vi "Toast With Reply.vi"(8 "error in":errorcluster) -> (0 "error out":errorcluster, 3 "Toast XML":string)   [LabVIEW 2026]
doc: "Receive a text reply from a Windows toast as a LabVIEW User Event. Type a reason, click Send and inspect the Reason entry in Activation.User Inputs. An empty reply still returns the Reason key. Press Stop to close the example."
uses:
  ToastNotification/Activation.ctl
  ToastNotification/Argument.ctl
  PlugIns/UserEventActivationHandler/UserEventActivationHandler.lvclass
  PlugIns/UserEventActivationHandler/UserEventActivationHandler.lvclass/UserEventActivationHandler.ctl
  PlugIns/UserEventActivationHandler/Read Event Ref.vi
  ToastBuilder/ToastBuilder.lvclass
  ToastBuilder/Create ToastBuilder.vi
  ToastService/ToastService.lvclass
  ToastNotification/ToastNotification.lvlib
panel:
  out "error":errorcluster
  out "Activation":T1
  in  "stop":bool
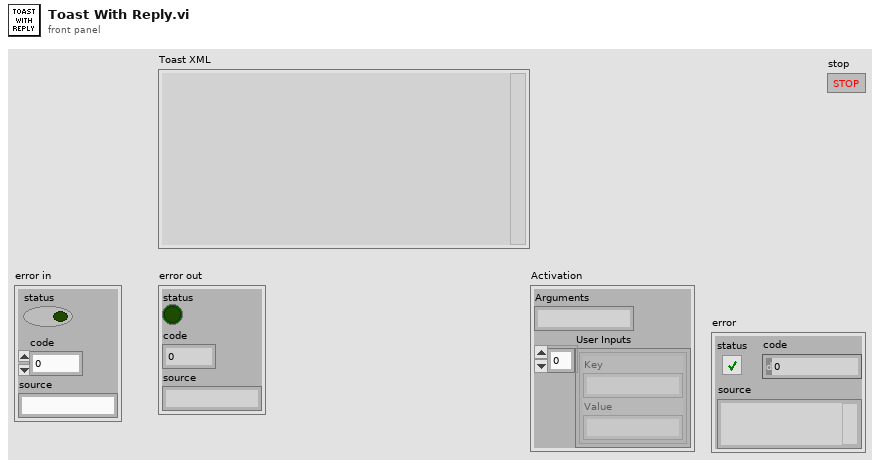
[diagram p1: front panel]
types:
  T1 = typedef "ToastNotification.lvlib/Activation.ctl" = cluster{"Arguments":string, "User Inputs":T2[]}
  T2 = typedef "ToastNotification.lvlib/Argument.ctl" = cluster{"Key":string, "Value":string}
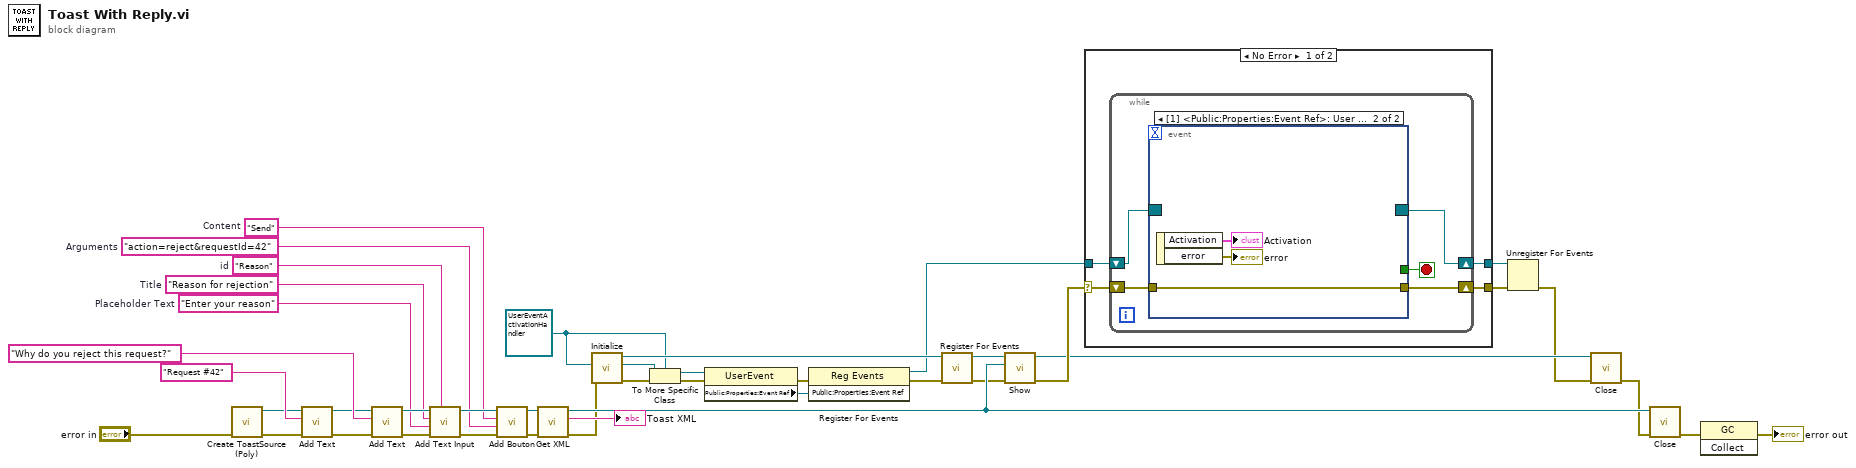
[diagram p0: block diagram]
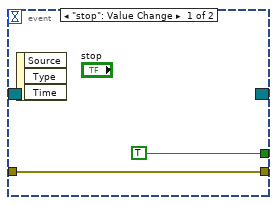
[diagram p2: hidden frame]
diagram:
  w14 = "action=reject&requestId=42"  # Arguments
  w15 = "Send"  # Content
  w20 = "Enter your reason"  # Placeholder Text
  w21 = "Reason for rejection"  # Title
  w22 = "Reason"  # id
  w12 = refnum<class "UserEventActivationHandler.lvclass"> refnum
  n1 = call-poly "Create ToastSource (Poly).vi"("error in"="error in") -> ("error out"=w36:errorcluster, "ToastBuilder out"=w35:refnum<class "ToastBuilder.lvclass">)  [unwired: 9 in]
  n2 = call "Add Text.vi"("error in"=w36, "text"="Request #42", "ToastBuilder in"=w35) -> ("error out"=w39:errorcluster, "ToastBuilder out"=w38:refnum<class "ToastBuilder.lvclass">)  [unwired: 7 in]
  n3 = call "Add Text.vi"("error in"=w39, "text"="Why do you reject this request?", "ToastBuilder in"=w38) -> ("error out"=w23:errorcluster, "ToastBuilder out"=w24:refnum<class "ToastBuilder.lvclass">)  [unwired: 7 in]
  n4 = call "Add Text Input.vi"("id"=w22, "error in (no error)"=w23, "Placeholder Text"=w20, "Title"=w21, "ToastBuilder in"=w24) -> ("error out"=w19:errorcluster, "ToastBuilder out"=w17:refnum<class "ToastBuilder.lvclass">)  [unwired: 5 in]
  n5 = call "Add Bouton.vi"("error in (no error)"=w19, "Arguments"=w14, "Content"=w15, "ToastBuilder in"=w17) -> ("error out"=w18:errorcluster, "ToastBuilder out"=w16:refnum<class "ToastBuilder.lvclass">)  [unwired: 6 in]
  n6 = call-dynamic "Get XML.vi"("error in"=w18, "ToastBuilder in"=w16) -> ("error out"=w32:errorcluster, "GetContent"=→"Toast XML":string, "ToastBuilder out"=w33:refnum<class "ToastBuilder.lvclass">)  [unwired: 7 in]
  n7 = call "Initialize.vi"("error in (no error)"=w32, "ActivationHandler in"=w12) -> ("error out"=w30:errorcluster, "ActivationHandler out"=w11:refnum<class "UserEventActivationHandler.lvclass">, "ToastService out"=w29:refnum<class "ToastService.lvclass">)  [unwired: 7 in]
  n8 = To More Specific Class(target class=w12, reference=w11, error in=w30) -> (specific class reference=w9:refnum<class "UserEventActivationHandler.lvclass">, error out=w13:errorcluster)
  n9 = property class="UserEvent"(reference=w9, error in=w13) -> (error out=w10:errorcluster, "Public:Properties:Event Ref"=w7:refnum<user-event>)  [unwired: 1 out]
  n10 = register-events(error in=w10, w7) -> (reference out=w3:refnum<event-registration>, error out=w8:errorcluster)  [unwired: 1 in]
  n11 = call "Register For Events.vi"("error in (no error)"=w8, "ToastService in"=w29) -> ("error out"=w2:errorcluster, "ToastService out"=w1:refnum<class "ToastService.lvclass">)  [unwired: 8 in]
  n12 = call "Show.vi"("error in (no error)"=w2, "ToastSource in"=w33, "ToastService in"=w1) -> ("error out"=w28:errorcluster, "ToastService out"=w27:refnum<class "ToastService.lvclass">)  [unwired: 7 in]
  n13 = case shown="No Error" w28 {
    selector: w28 -> [w45 w56]
    tunnel: [w44 w56] -> w6
    tunnel: w3 -> [w43 w57]
    tunnel: [w42 w57] -> w4
    frame No Error {
      n14 = while {
        shift-right: [w49] -> w44
        shift-left: w45 -> [w50]
        shift-right: [w47] -> w42
        shift-left: w43 -> [w48]
        stop <- w46 stop-if-true
        n15 = event shown="[1] <Public:Properties:Event Ref>: User Event" {
          selector: w48 -> [_ _]
          dyn-events: [_ _] -> w47
          timeout: _ -> [_ _]
          tunnel: [w52 w55] -> w49
          tunnel: w50 -> [w52 w55]
          tunnel: [TRUE _] -> w46
          event "stop": Value Change {
            n16 = event-data() -> ()  [unwired: 1 in, 3 out]
          }
          event User Event {
            n17 = event-data() -> ("Activation"=→"Activation":T1, "error"=→"error":errorcluster)  [unwired: 1 in]
          }
        }
      }
    }
    frame Error {
    }
  }
  n18 = Unregister For Events(event registration refnum=w4, error in=w6) -> (error out=w5:errorcluster)
  n19 = call "Close.vi"("error in (no error)"=w5, "ToastService in"=w27) -> ("error out"=w31:errorcluster)  [unwired: 9 in]
  n20 = call-dynamic "Close.vi"("error in"=w31, "ToastBuilder in"=w33) -> ("error out"=w26:errorcluster)  [unwired: 9 in]
  n21 = invoke class="GC" method="Collect"(error in=w26) -> (error out=→"error out":errorcluster)  [unwired: 2 in, 2 out]
